vi "get all control details.vi"(8 "error in":errorcluster, 11 "VI (Caller)":refnum<vi>) -> (0 "error out":errorcluster, 3 "Control details":string)   [LabVIEW 2020, in "ui-testing.lvlib"]
uses:
  ui-testing.lvlib
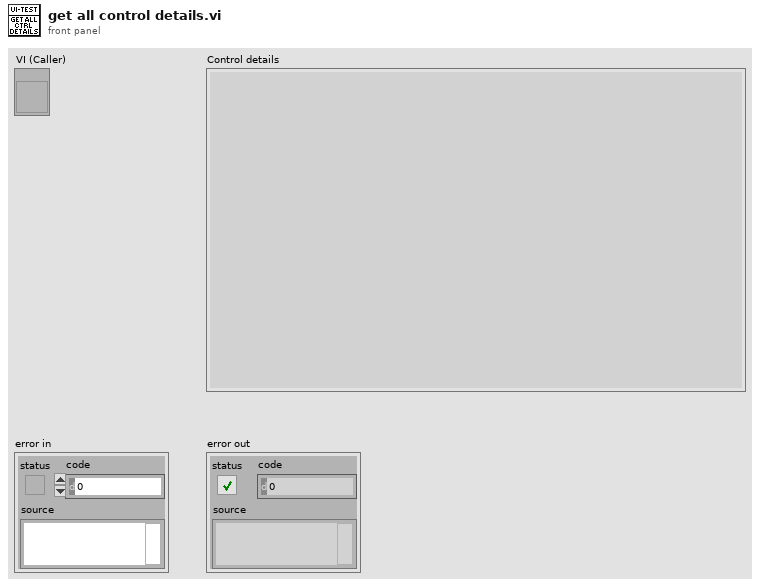
[diagram p1: front panel]
types:
  T1 = cluster{"Caption":string, "Label":string, "Visible":bool}
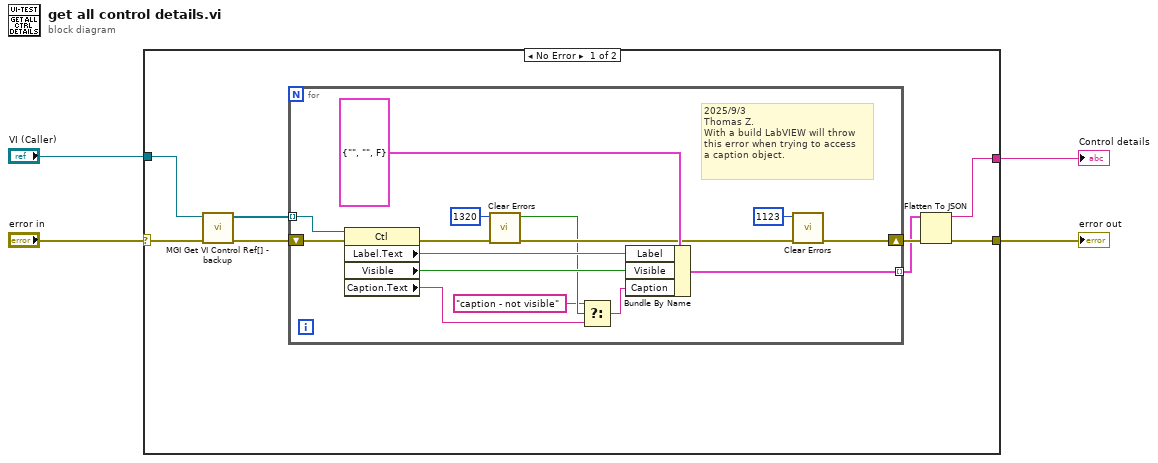
[diagram p0: block diagram]
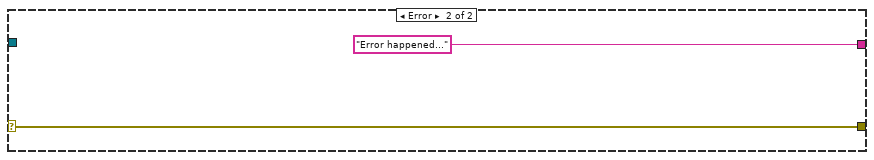
[diagram p2: hidden frame]
diagram:
  n1 = case shown="No Error" "error in" {
    selector: "error in" -> [w5 w29]
    tunnel: [w9 w29] -> w4
    tunnel: [w7 "Error happened..."] -> w3
    tunnel: "VI (Caller)" -> [w6 _]
    frame No Error {
      n2 = call "MGI Get VI Control Ref[] - backup.vi"("error in"=w5, "VI (Caller)"=w6) -> ("error out"=w12:errorcluster, "Control[i]"=w11:refnum<vi>[])  [unwired: 6 in, 2 out]
      n3 = for {
        tunnel: w11 -> [w26] mode=indexing
        tunnel: [w22] -> w8 mode=indexing
        shift-right: [w14] -> w10
        shift-left: w12 -> [w27]
        # "2025/9/3\nThomas Z.\nWith a build LabVIEW will throw\nthis error when trying to access\na caption object."
        n4 = property class="Ctl"(reference=w26, error in=w27) -> (error out=w21:errorcluster, "Label.Text"=w25:string, "Visible"=w24:bool, "Caption.Text"=w18:string)  [unwired: 1 out]
        n5 = call <vilib>:"Clear Errors.vi"("error in (no error)"=w21, "specific error code to clear (0: all)"=1320) -> ("error out"=w20:errorcluster, "specific error cleared?"=w16:bool)  [unwired: 4 in]
        n6 = Select(t="caption - not visible", s=w16, f=w18) -> (s? t:f=w17:string)
        n7 = Bundle By Name(cluster=T1 {"Caption"="", "Label"="", "Visible"=FALSE}, "Label"=w25, "Visible"=w24, "Caption"=w17) -> (w22:T1)
        n8 = call <vilib>:"Clear Errors.vi"("error in (no error)"=w20, "specific error code to clear (0: all)"=1123) -> ("error out"=w14:errorcluster)  [unwired: 4 in, 1 out]
      }
      n9 = Flatten To JSON(anything=w8, error in (no error)=w10) -> (JSON string=w7:string, 11:w9:errorcluster)  [unwired: 1 in]
    }
    frame Error {
    }
  }
  "error out" <- w4
  "Control details" <- w3
